vi "Voltage_output.vi"(1 "Feedback enabled?":refnum<vi>, 2 "Iteration count":refnum<vi>, 6 "Current Motion":T1, 8 "Updated Motion Output Row":refnum<vi>, 9 "Current Motion Output":T2, 10 "Instant Start / Stop":refnum<vi>, 11 "Toggle IN":bool) -> (3 "Toggle OUT":bool)   [LabVIEW 2019]
uses:
  Type_definition_current_motion.ctl
  <vilib>/DAQmx/write.llb/DAQmx Write (Analog 1D DBL NChan 1Samp).vi
  <vilib>/DAQmx/write.llb/DAQmx Write (Digital 1D Bool 1Chan 1Samp).vi
  <vilib>/DAQmx/create/channels.llb/DAQmx Create Channel (AO-Voltage-Basic).vi
  <vilib>/DAQmx/create/channels.llb/DAQmx Create Channel (DO-Digital Output).vi
  <vilib>/DAQmx/miscellaneous.llb/DAQmx Fill In Error Info.vi
panel:
  out "loop time":u32
  out "Iteration":i32
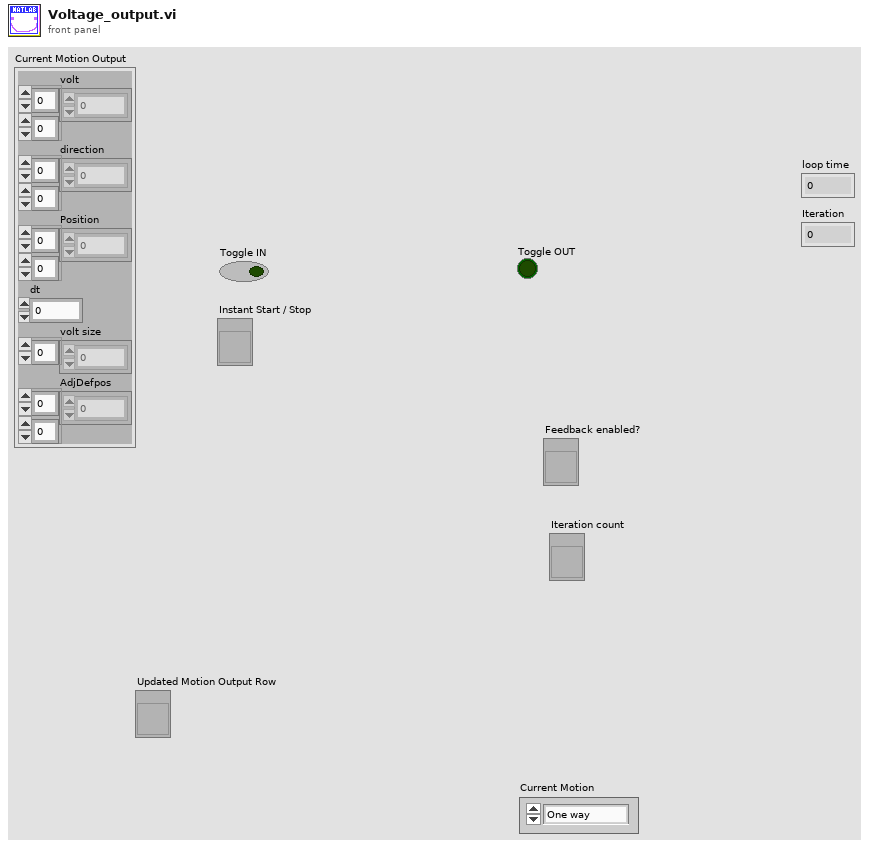
[diagram p1: front panel]
types:
  T1 = typedef "Type_definition_current_motion.ctl" = enum16{"One way", "Rot", "Tilt", "Tau", "XYZrot", "Zvert", "YZcirc", "Random direction tilt"}
  T2 = cluster{"volt":dbl[][], "direction":dbl[][], "Position":dbl[][], "dt":dbl, "volt size":i32[], "AdjDefpos":dbl[][]}
  T3 = cluster{"For Iteration":dbl, "Updated volt":dbl[][], "Updated direction":dbl[][], "Posoffset":dbl[][], "For Motion":T1}
  T4 = cluster{"volt 1,2":dbl[], "volt 3,4":dbl[], "volt 5,6":dbl[]}
  T5 = cluster{"digital 1,2":bool[], "digital 3,4":bool[], "digital 5,6":bool[]}
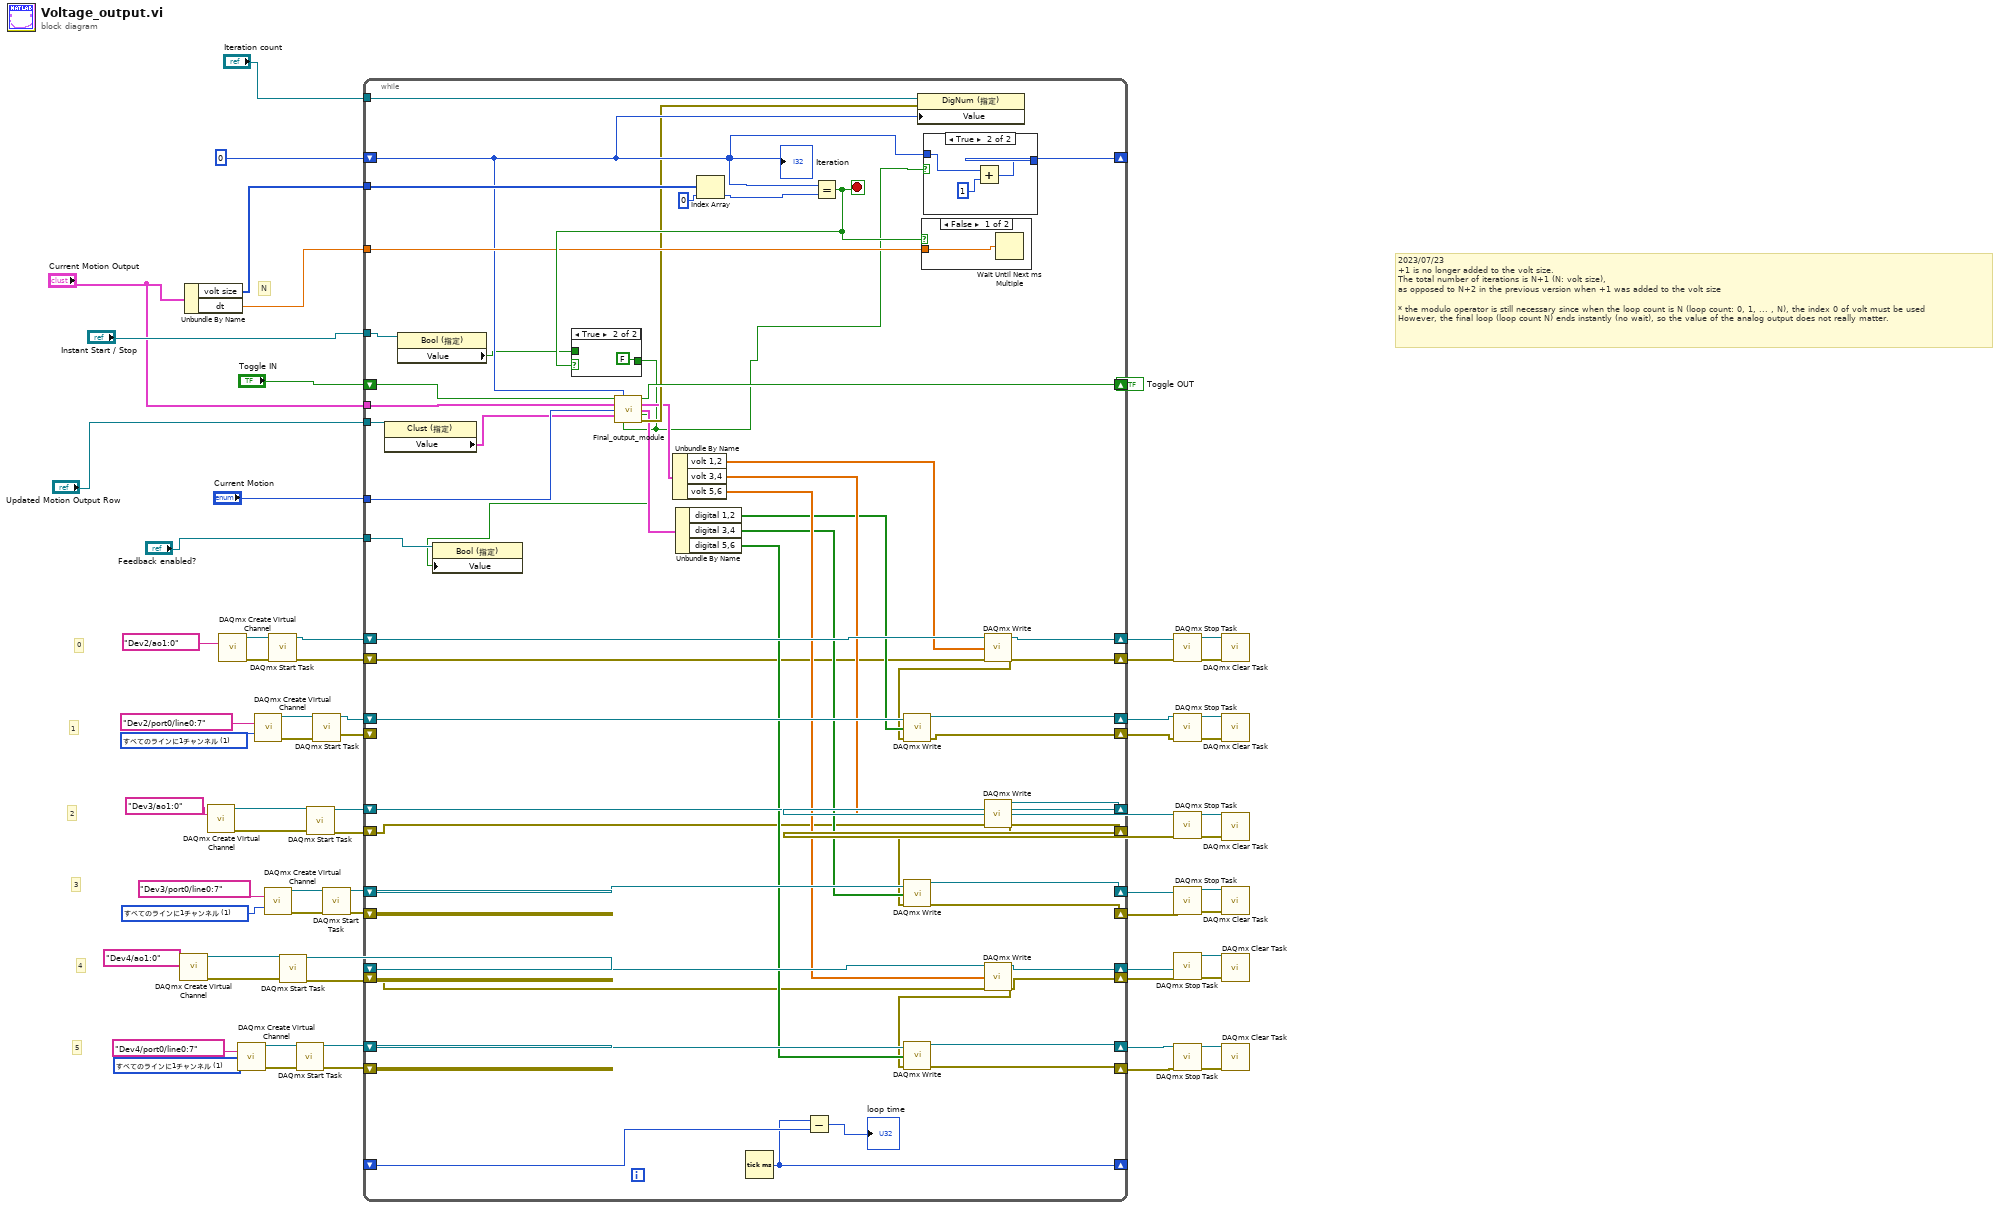
[diagram p0: block diagram]
diagram:
  w36 = 1 items=["各ラインに1チャンネル", "すべてのラインに1チャンネル"] ("line grouping")
  w42 = 1 items=["各ラインに1チャンネル", "すべてのラインに1チャンネル"] ("line grouping")
  w54 = 1 items=["各ラインに1チャンネル", "すべてのラインに1チャンネル"] ("line grouping")
  # "N"
  # "5"
  # "4"
  # "3"
  # "2"
  # "1"
  # "0"
  # "2023/07/23\n+1 is no longer added to the volt size. \nThe total number of iterations is N+1 (N: volt size), \nas opposed to N+2 in the previous version when +1 was added to the volt size\n\n* the modulo operator is still necessary since when the loop count is N (loop count: 0, 1, ... , N), the index 0 of volt must be used\nHowever, the final loop (loop count N) ends instantly (no wait), so the value of the analog output does not really matter."
  n1 = call-poly <vilib>:"DAQmx Create Virtual Channel.vi"("physical channels"=tag "Dev4/ao1:0") -> ("task out"=w31:refnum<k21>, "error out"=w30:errorcluster)  [unwired: 13 in]
  n2 = Unbundle By Name("Current Motion Output") -> ("volt size"=w68:i32[], "dt"=w67:dbl)
  n3 = call-poly <vilib>:"DAQmx Create Virtual Channel.vi"("physical channels"=tag "Dev3/ao1:0") -> ("task out"=w59:refnum<k21>, "error out"=w60:errorcluster)  [unwired: 13 in]
  n4 = call-poly <vilib>:"DAQmx Create Virtual Channel.vi"("physical channels"=tag "Dev2/ao1:0") -> ("task out"=w50:refnum<k21>, "error out"=w49:errorcluster)  [unwired: 13 in]
  n5 = call-poly <vilib>:"DAQmx Create Virtual Channel.vi"("lines"=tag "Dev4/port0/line0:7", "line grouping"=w36) -> ("task out"=w33:refnum<k21>, "error out"=w34:errorcluster)  [unwired: 12 in]
  n6 = call-poly <vilib>:"DAQmx Create Virtual Channel.vi"("lines"=tag "Dev2/port0/line0:7", "line grouping"=w42) -> ("task out"=w39:refnum<k21>, "error out"=w40:errorcluster)  [unwired: 12 in]
  n7 = call-poly <vilib>:"DAQmx Create Virtual Channel.vi"("lines"=tag "Dev3/port0/line0:7", "line grouping"=w54) -> ("task out"=w57:refnum<k21>, "error out"=w56:errorcluster)  [unwired: 12 in]
  n8 = call <vilib>:"DAQmx Start Task.vi"("task/channels in"=w50, "error in"=w49) -> ("task out"=w46:refnum<k21>, "error out"=w45:errorcluster)  [unwired: 12 in]
  n9 = call <vilib>:"DAQmx Start Task.vi"("task/channels in"=w31, "error in"=w30) -> ("task out"=w27:refnum<k21>, "error out"=w26:errorcluster)  [unwired: 12 in]
  n10 = call <vilib>:"DAQmx Start Task.vi"("task/channels in"=w33, "error in"=w34) -> ("task out"=w23:refnum<k21>, "error out"=w22:errorcluster)  [unwired: 12 in]
  n11 = call <vilib>:"DAQmx Start Task.vi"("task/channels in"=w59, "error in"=w60) -> ("task out"=w61:refnum<k21>, "error out"=w62:errorcluster)  [unwired: 12 in]
  n12 = call <vilib>:"DAQmx Start Task.vi"("task/channels in"=w39, "error in"=w40) -> ("task out"=w38:refnum<k21>, "error out"=w37:errorcluster)  [unwired: 12 in]
  n13 = call <vilib>:"DAQmx Start Task.vi"("task/channels in"=w57, "error in"=w56) -> ("task out"=w53:refnum<k21>, "error out"=w52:errorcluster)  [unwired: 12 in]
  n14 = while {
    shift-right: [w119] -> w63
    shift-left: w61 -> [w120]
    shift-right: [w72] -> w64
    shift-left: w62 -> [w73]
    shift-right: [w117] -> w15
    shift-left: w53 -> [w118]
    shift-right: [w98] -> w14
    shift-left: w52 -> [_]
    shift-right: [w116] -> _
    shift-left: 0 -> [w93]
    shift-right: [w113] -> w44
    shift-left: w46 -> [w114]
    shift-right: [w74] -> w43
    shift-left: w45 -> [w75]
    shift-right: [w111] -> w19
    shift-left: w38 -> [w112]
    shift-right: [w99] -> w18
    shift-left: w37 -> [_]
    shift-right: [w109] -> w25
    shift-left: w27 -> [w110]
    shift-right: [w70] -> w24
    shift-left: w26 -> [w71]
    shift-right: [w107] -> w11
    shift-left: w23 -> [w108]
    shift-right: [w97] -> w10
    shift-left: w22 -> [_]
    shift-right: [w105] -> _
    shift-left: _ -> [w106]
    tunnel: w68 -> [w102]
    tunnel: w67 -> [w101]
    tunnel: "Instant Start / Stop" -> [w100]
    tunnel: "Iteration count" -> [w96]
    tunnel: "Current Motion Output" -> [w94]
    tunnel: "Updated Motion Output Row" -> [w77]
    shift-right: [w92] -> w6
    shift-left: "Toggle IN" -> [w91]
    tunnel: "Current Motion" -> [w90]
    tunnel: "Feedback enabled?" -> [w79]
    stop <- w103 stop-if-true
    n15 = property class="Clust (指定)"(reference=w77) -> ("Value"=w76:T3)  [unwired: 1 in, 2 out]
    n16 = property class="Bool (指定)"(reference=w100) -> ("Value"=w89:bool)  [unwired: 1 in, 2 out]
    n17 = Index Array(array=w102, index=0) -> (element=w95:i32)
    n18 = Tick Count (ms)() -> (millisecond timer value=w105:u32)
    n19 = Subtract(x=w105, y=w106) -> (x-y=→"loop time":u32)
    n20 = Equal?(x=w93, y=w95) -> (x = y?=w103:bool)
    n21 = case shown="TRUE" w103 {
      tunnel: [w126 FALSE] -> w69
      tunnel: w89 -> [w126 _]
      frame False {
      }
      frame True {
      }
    }
    n22 = call "Final_output_module.vi"("Toggle IN"=w91, "Iteration"=w93, "Current Motion Output"=w94, "Current Motion"=w90, "Updated Motion Output Row"=w76, "Instant start/stop 0 to 1"=w69) -> ("Toggle OUT"=w92:bool, "volt cluster"=w87:T4, "digital cluster"=w85:T5, "Feedback enabled?"=w78:bool, "Error OUT"=w88:errorcluster)  [unwired: 5 in]
    n23 = property class="Bool (指定)"(reference=w79, "Value"=w78) -> ()  [unwired: 1 in, 2 out]
    n24 = Unbundle By Name(w87) -> ("volt 1,2"=w86:dbl[], "volt 3,4"=w84:dbl[], "volt 5,6"=w83:dbl[])
    n25 = Unbundle By Name(w85) -> ("digital 1,2"=w82:bool[], "digital 3,4"=w81:bool[], "digital 5,6"=w80:bool[])
    n26 = property class="DigNum (指定)"(reference=w96, error in=w88, "Value"=w93) -> ()  [unwired: 2 out]
    n27 = case shown="FALSE" w103 {
      tunnel: w101 -> [w121 _]
      frame False {
        n28 = Wait Until Next ms Multiple(millisecond multiple=w121) -> ()  [unwired: 1 out]
      }
      frame True {
      }
    }
    n29 = case shown="TRUE" w69 {
      tunnel: [w122 w125] -> w116
      tunnel: w93 -> [w122 w123]
      frame False {
      }
      frame True {
        n30 = Add(x=w123, y=1) -> (x+y=w125:i32)
      }
    }
    n31 = call-poly <vilib>:"DAQmx Write.vi"("task/channels in"=w114, "data"=w86, "error in"=w75) -> ("task out"=w113:refnum<k21>, "error out"=w74:errorcluster)  [unwired: 10 in, 1 out]
    n32 = call-poly <vilib>:"DAQmx Write.vi"("task/channels in"=w112, "data"=w82, "error in"=w74) -> ("task out"=w111:refnum<k21>, "error out"=w99:errorcluster)  [unwired: 10 in, 1 out]
    n33 = call-poly <vilib>:"DAQmx Write.vi"("task/channels in"=w120, "data"=w84, "error in"=w73) -> ("task out"=w119:refnum<k21>, "error out"=w72:errorcluster)  [unwired: 10 in, 1 out]
    n34 = call-poly <vilib>:"DAQmx Write.vi"("task/channels in"=w118, "data"=w81, "error in"=w72) -> ("task out"=w117:refnum<k21>, "error out"=w98:errorcluster)  [unwired: 10 in, 1 out]
    n35 = call-poly <vilib>:"DAQmx Write.vi"("task/channels in"=w110, "data"=w83, "error in"=w71) -> ("task out"=w109:refnum<k21>, "error out"=w70:errorcluster)  [unwired: 10 in, 1 out]
    n36 = call-poly <vilib>:"DAQmx Write.vi"("task/channels in"=w108, "data"=w80, "error in"=w70) -> ("task out"=w107:refnum<k21>, "error out"=w97:errorcluster)  [unwired: 10 in, 1 out]
    "Iteration" <- w93
  }
  "Toggle OUT" <- w6
  n37 = call <vilib>:"DAQmx Stop Task.vi"("task/channels in"=w44, "error in"=w43) -> ("task out"=w48:refnum<k21>, "error out"=w47:errorcluster)  [unwired: 12 in]
  n38 = call <vilib>:"DAQmx Stop Task.vi"("task/channels in"=w19, "error in"=w18) -> ("task out"=w21:refnum<k21>, "error out"=w20:errorcluster)  [unwired: 12 in]
  n39 = call <vilib>:"DAQmx Stop Task.vi"("task/channels in"=w63, "error in"=w64) -> ("task out"=w65:refnum<k21>, "error out"=w66:errorcluster)  [unwired: 12 in]
  n40 = call <vilib>:"DAQmx Stop Task.vi"("task/channels in"=w15, "error in"=w14) -> ("task out"=w16:refnum<k21>, "error out"=w17:errorcluster)  [unwired: 12 in]
  n41 = call <vilib>:"DAQmx Stop Task.vi"("task/channels in"=w25, "error in"=w24) -> ("task out"=w29:refnum<k21>, "error out"=w28:errorcluster)  [unwired: 12 in]
  n42 = call <vilib>:"DAQmx Stop Task.vi"("task/channels in"=w11, "error in"=w10) -> ("task out"=w13:refnum<k21>, "error out"=w12:errorcluster)  [unwired: 12 in]
  n43 = call <vilib>:"DAQmx Clear Task.vi"("task in"=w48, "error in"=w47) -> ()  [unwired: 13 in, 1 out]
  n44 = call <vilib>:"DAQmx Clear Task.vi"("task in"=w21, "error in"=w20) -> ()  [unwired: 13 in, 1 out]
  n45 = call <vilib>:"DAQmx Clear Task.vi"("task in"=w65, "error in"=w66) -> ()  [unwired: 13 in, 1 out]
  n46 = call <vilib>:"DAQmx Clear Task.vi"("task in"=w16, "error in"=w17) -> ()  [unwired: 13 in, 1 out]
  n47 = call <vilib>:"DAQmx Clear Task.vi"("task in"=w29, "error in"=w28) -> ()  [unwired: 13 in, 1 out]
  n48 = call <vilib>:"DAQmx Clear Task.vi"("task in"=w13, "error in"=w12) -> ()  [unwired: 13 in, 1 out]
